vi "Timestamp to ISO8601 Time.vi"(5 "Delimiter (system)":T1, 6 "T Delimiter? (T)":bool=TRUE, 7 "Unit (ms)":T2=enum."millisecond", 9 "UTC? (F)":bool, 11 "Timestamp (now)":timestamp) -> (3 "ISO8601 Time":string)   [LabVIEW 2013]
doc: "Converts a <b>Timestamp</b> to <b>ISO8601 Time</b> string without time zone designator.\n\n<b>UTC?:</b> True: Time in Coordinated Universal Time. False (default): Time in user's local time zone.\n\n<b>\"T\" delimiter?:</b> ISO8601 requires a leading 'T' delimiter to lift ambiguity; default is True.\n\n<b>Units</b>: Seconds field precision; default is milliseconds."
uses:
  Seconds Units -- enum.ctl
  Locale -- enum.ctl
  Epoch_NotationLocale.vi
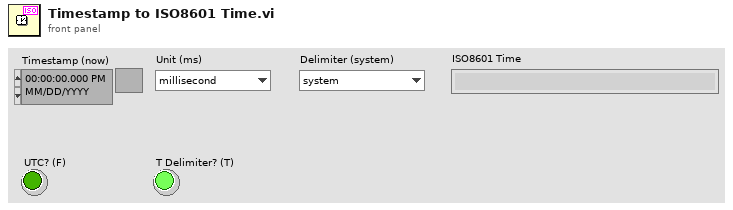
[diagram p1: front panel]
types:
  T1 = typedef "Locale -- enum.ctl" = enum16{"system", "Dot notation", "Comma notation", "custom"}
  T2 = typedef "Seconds Units -- enum.ctl" = enum16{"second", "millisecond", "microsecond", "nanosecond"}
  T3 = typedef "LVDateTimeRec.ctl" = cluster{"fractional second":dbl, "second":i32, "minute":i32, "hour":i32, "day of month":i32, "month":i32, "year":i32, "day of week":i32, "day of year":i32, "DST":i32}
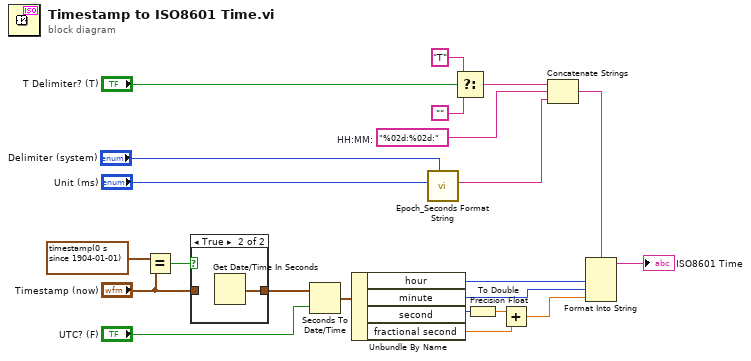
[diagram p0: block diagram]
diagram:
  w9 = "%02d:%02d:"  # HH:MM:
  n1 = Equal?(x=timestamp(0 s since 1904-01-01), y="Timestamp (now)") -> (x = y?=w18:bool)
  n2 = case shown="True" w18 {
    tunnel: [w23 w24] -> w2
    tunnel: "Timestamp (now)" -> [w23 _]
    frame False {
    }
    frame True {
      n3 = Get Date/Time In Seconds() -> (seconds since 1Jan1904=w24:timestamp)
    }
  }
  n4 = Seconds To Date/Time(time stamp (now)=w2, to UTC (F)="UTC? (F)") -> (date time rec=w20:T3)
  n5 = Unbundle By Name(w20) -> ("hour"=w16:i32, "minute"=w15:i32, "second"=w8:i32, "fractional second"=w7:dbl)
  n6 = call "Epoch_Seconds Format String.vi"("Delimiter (system)"="Delimiter (system)", "Unit (ms)"="Unit (ms)") -> ("format string"=w4:string)  [unwired: 9 in]
  n7 = Select(t="T", s="T Delimiter? (T)", f="") -> (s? t:f=w12:string)
  n8 = To Double Precision Float(number=w8) -> (double precision float=w3:dbl)
  n9 = Add(x=w3, y=w7) -> (x+y=w6:dbl)
  n10 = Concatenate Strings(w12, w9, w4) -> (w13:string)
  n11 = Format Into String(format string=w13, w16, w15, w6) -> (resulting string=→"ISO8601 Time":string)  [unwired: 2 in, 1 out]
